vi "Test Helper Loop Multiple Parallell Helper Loops.vi"(8 "error in (no error)":errorcluster, 11 "Helper Loop Test In":refnum<class "Helper Loop Test.lvclass">) -> (0 "error out":errorcluster, 3 "Helper Loop Test Out":refnum<class "Helper Loop Test.lvclass">)   [LabVIEW 2020, in "Helper Loop Test.lvclass"]
uses:
  Helper Loop Test.lvclass
  C:/Program Files (x86)/National Instruments/LabVIEW 2020/vi.lib/Astemes/LUnit/Test Case.lvclass
  source/Framework Test Suite/Mock Process/Mock Process.lvclass
  C:/git/astemes-triarc-framework/source/Framework/Process/Process.lvclass
  <vilib>/Astemes/LUnit/Test Case.lvclass/Test Case.ctl
  source/Framework/Process/Process.lvclass/Process.ctl
  50b6e122-0124-4b7b-aa32-eb2a86067106.vi
  42738f38-96e3-4277-8aab-a77fd84bb115.vi
  source/Framework/Broadcast Event Dequeuers/Execution timer.vi
  <vilib>/Astemes/LUnit/Append Pass Result.vi
  <vilib>/Astemes/LUnit/Append Fail Result.vi
  50b6e122-0124-4b7b-aa32-eb2a86067106.vi/9c5d11cd-9439-4240-a1ee-d9baace9c924.vi
  source/Framework/Process/Private/SubVIs/Wait for finish.vi
  source/Framework/Process/Private/SubVIs/Set Lifecycle State.vi
  source/Framework/Process/Protected/Messaging/Send Message.vi
  42738f38-96e3-4277-8aab-a77fd84bb115.vi/9c5d11cd-9439-4240-a1ee-d9baace9c924.vi
  <vilib>/Astemes/LUnit/Run In UI.vi
  source/Framework/Process/Private/SubVIs/Handle Debug Data.vi
  <vilib>/Utility/error.llb/Clear Errors.vi
  source/Framework/Logging/Log Debug.vi
  <vilib>/AdvancedString/1D String Array to Delimited String.vi
  <vilib>/Utility/High Resolution Relative Seconds.vi
  source/Framework/Broadcast Event Dequeuers/Dequeue Broadcast Message.vi
  source/Framework/Process/Public/Lifecycle/Get Lifecycle State.vi
  <vilib>/Utility/error.llb/Error Cluster From Error Code.vi
  source/Framework/Process/Public/Read Name.vi
  source/Framework/Callback/Callback.lvclass
  source/Framework/Process/Process.lvclass
  Helper Loop Test.lvclass/Helper Loop Test.ctl
  source/Framework/Broadcast Event Dequeuers/Broadcast Event Dequeuers.lvlib
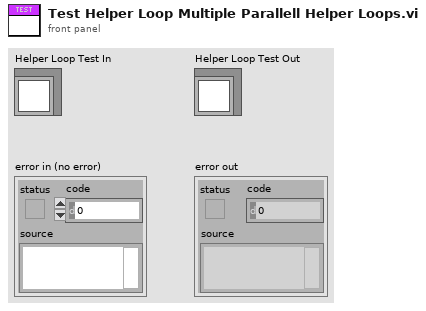
[diagram p1: front panel]
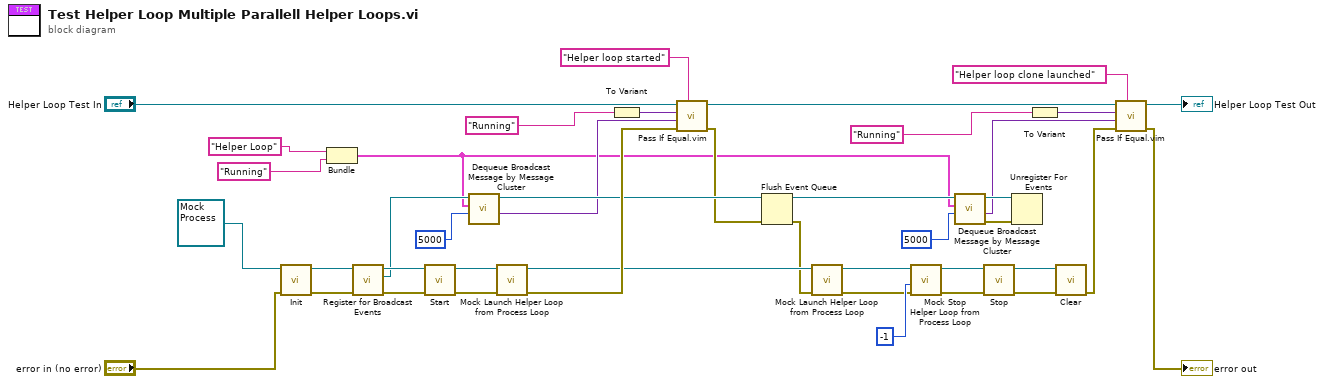
[diagram p0: block diagram]
diagram:
  n1 = call-dynamic "Init.vi"("error in (no error)"="error in (no error)", "Mock Process In"=refnum<class "Mock Process.lvclass"> refnum) -> ("error out"=w42:errorcluster, "Mock Process Out"=w22:refnum<class "Mock Process.lvclass">)  [unwired: 8 in]
  n2 = Bundle("y"="Helper Loop", "Description"="Running") -> (w3:cluster{"y":string, "Description":string})  [unwired: 1 in]
  n3 = call "Register for Broadcast Events.vi"("error in (no error)"=w42, "Process In"=w22) -> ("error out"=w23:errorcluster, "Event Registration Refnum Out"=w18:refnum<event-registration>, "Process Out"=w21:refnum<class "Mock Process.lvclass">)  [unwired: 7 in]
  n4 = call "Start.vi"("error in (no error)"=w23, "Process In"=w21) -> ("error out"=w40:errorcluster, "Process Out"=w41:refnum<class "Mock Process.lvclass">)  [unwired: 7 in, 1 out]
  n5 = call "Dequeue Broadcast Message by Message Cluster.vi"("Timeout (-1)"=5000, "Message"=w3, "Event Registration Refnum"=w18) -> ("Message Data"=w7:variant, "Event Registration Refnum Out"=w15:refnum<event-registration>)  [unwired: 4 in, 3 out]
  n6 = call "Mock Launch Helper Loop from Process Loop.vi"("error in (no error)"=w40, "Mock Process in"=w41) -> ("error out"=w29:errorcluster, "Mock Process out"=w28:refnum<class "Mock Process.lvclass">)  [unwired: 8 in]
  n7 = To Variant(anything="Running") -> (Variant=w1:variant)
  n8 = call "Pass If Equal.vim"("Description"="Helper loop started", "error in (no error)"=w29, "Actual"=w7, "Expected"=w1, "LUnit Test Case In"="Helper Loop Test In") -> ("error out"=w14:errorcluster, "LUnit Test Case Out"=w31:refnum<class "Helper Loop Test.lvclass">)  [unwired: 5 in]
  n9 = Flush Event Queue(0:w15, 3:w14) -> (8:w12:refnum<event-registration>, 11:w13:errorcluster)  [unwired: 4 in, 1 out]
  n10 = call "Mock Launch Helper Loop from Process Loop.vi"("error in (no error)"=w13, "Mock Process in"=w28) -> ("error out"=w19:errorcluster, "Mock Process out"=w20:refnum<class "Mock Process.lvclass">)  [unwired: 8 in]
  n11 = call "Mock Stop Helper Loop from Process Loop.vi"("error in (no error)"=w19, "timeout in ms (-1)"=-1, "Mock Process in"=w20) -> ("error out"=w26:errorcluster, "Mock Process out"=w27:refnum<class "Mock Process.lvclass">)  [unwired: 6 in, 1 out]
  n12 = call "Dequeue Broadcast Message by Message Cluster.vi"("Timeout (-1)"=5000, "Message"=w3, "Event Registration Refnum"=w12) -> ("error out"=w9:errorcluster, "Message Data"=w6:variant, "Event Registration Refnum Out"=w8:refnum<event-registration>)  [unwired: 4 in, 2 out]
  n13 = call "Stop.vi"("error in (no error)"=w26, "Process In"=w27) -> ("error out"=w39:errorcluster, "Process Out"=w24:refnum<class "Mock Process.lvclass">)  [unwired: 7 in, 1 out]
  n14 = Unregister For Events(event registration refnum=w8, error in=w9) -> ()  [unwired: 1 out]
  n15 = To Variant(anything="Running") -> (Variant=w2:variant)
  n16 = call-dynamic "Clear.vi"("error in (no error)"=w39, "Mock Process In"=w24) -> ("error out"=w38:errorcluster)  [unwired: 9 in]
  n17 = call "Pass If Equal.vim"("Description"="Helper loop clone launched", "error in (no error)"=w38, "Actual"=w6, "Expected"=w2, "LUnit Test Case In"=w31) -> ("error out"=→"error out":errorcluster, "LUnit Test Case Out"=→"Helper Loop Test Out":refnum<class "Helper Loop Test.lvclass">)  [unwired: 5 in]
